vi "VHist - Multiple DBL history to Table.vi"(4 "data format (%.3f)":string="%.3f", 6 "time stamp format (%c)":string="%c", 7 "transpose (F)":bool, 8 "error in":errorcluster, 9 "empty for NaN (F)":bool, 10 "multiple history data":cluster{"history data":dbl[]}[](array[cluster]), 11 "time stamps":dbl[](array[numeric]) format="%<%H:%M:%S%2u\n%d/%m/%Y>T") -> (0 "error out":errorcluster, 2 "table data":string[][](array[string]), 3 "time stamp headers":string[](array[string]))   [LabVIEW 2021]
doc: "The VI converts multiple DBL history to 2D array of strings that can be displayed in a table. The VI returns time stamps in a separate 1D array of string that can be passed to a table header (e.g. row headers).\n\nIt is possible to specify format of numbers and time stamps. Optionally, the VI can replace NaN with an empty string, and transpose an output <table data> array.\n\n::: CalcExpress Toolkit :::\nCopyright (c) 2000-2026 Konstantin Shifershteyn. All rights reserved."
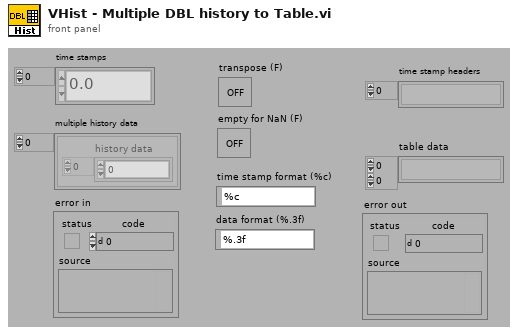
[diagram p1: front panel]
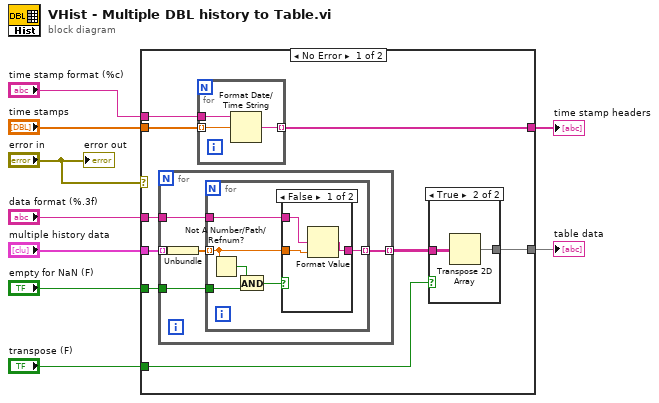
[diagram p0: block diagram]
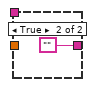
[diagram p3: hidden frame]
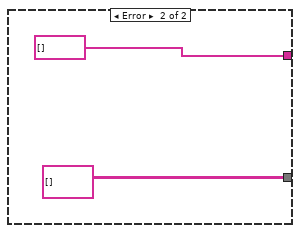
[diagram p4: hidden frame]
diagram:
  n1 = case shown="No Error" "error in" {
    tunnel: "time stamp format (%c)" -> [w18 _]
    tunnel: "time stamps" -> [w17 _]
    tunnel: "multiple history data" -> [w16 _]
    tunnel: "data format (%.3f)" -> [w15 _]
    tunnel: [w12 string[][] []] -> w4
    tunnel: [w14 string[] []] -> w5
    tunnel: "empty for NaN (F)" -> [w11 _]
    tunnel: "transpose (F)" -> [w10 _]
    frame No Error {
      n2 = for {
        tunnel: w16 -> [w29] mode=indexing
        tunnel: [w28] -> w13 mode=indexing
        tunnel: w15 -> [w26]
        tunnel: w11 -> [w25]
        n3 = Unbundle(w29) -> ("history data"=w27:dbl[])
        n4 = for {
          tunnel: [w35] -> w28 mode=indexing
          tunnel: w27 -> [w33] mode=indexing
          tunnel: w26 -> [w34]
          tunnel: w25 -> [w32]
          n5 = Not A Number/Path/Refnum?(number/path/refnum=w33) -> (NaN/Path/Refnum?=w31:bool)
          n6 = And(x=w31, y=w32) -> (x .and. y?=w30:bool)
          n7 = case shown="False" w30 {
            tunnel: [w38 ""] -> w35
            tunnel: w33 -> [w37 _]
            tunnel: w34 -> [w36 _]
            frame False {
              n8 = Format Value(format string=w36, value (0)=w37) -> (output string=w38:string)  [unwired: 1 in]
            }
            frame True {
            }
          }
        }
      }
      n9 = for {
        tunnel: w17 -> [w24] mode=indexing
        tunnel: w18 -> [w23]
        tunnel: [w22] -> w14 mode=indexing
        n10 = Format Date/Time String(time format string (%c)=w23, seconds (now)=w24) -> (date/time string=w22:string)  [unwired: 1 in]
      }
      n11 = case shown="True" w10 {
        tunnel: w13 -> [w19 w21]
        tunnel: [w19 w20] -> w12
        frame False {
        }
        frame True {
          n12 = Transpose 2D Array(2D array=w21) -> (transposed array=w20:string[][])
        }
      }
    }
    frame Error {
    }
  }
  "table data" <- w4
  "time stamp headers" <- w5
  "error out" <- "error in"
